vi "order-spectrum-flexlogger-test.vi"(1 "Order Settings":T2={"pulses per rev"=1, "trigger level (V)"=2.5, "max order"=64.0, "order resolution"=0.1, "window"=1, "averaging parameters"={"averaging mode"=enum."No averaging", "weighting mode"=enum."Linear", "number of averages"=1, "linear mode"=enum."One shot"}, "order ranges"=[{"start"=0.8, "stop"=1.2}, {"start"=1.8, "stop"=2.2}, {"start"=3.37, "stop"=3.77}, {"start"=3.8, "stop"=4.2}, {"start"=23.8, "stop"=24.2}]}, 4 "Noise (g rms)":dbl=0.01, 5 "Phases (deg)":dbl[](array[numeric])=[30.0, 0.0, 0.0, 0.0, 0.0], 6 "Orders":dbl[](array[numeric])=[1.0, 2.0, 3.57, 4.0, 24.0], 7 "Amplitudes (g pk)":dbl[](array[numeric])=[0.5, 0.2, 0.1, 0.05, 0.3], 8 "error in (no error)":errorcluster, 9 "Duration (s)":dbl=30.0, 10 "Ramps":T3(array[cluster]), 11 "Base RPM":dbl=3000.0) -> (0 "error out":errorcluster, 2 "True RPM":dbl[](array[numeric]), 3 "Tach RPM":dbl[](array[numeric]))   [LabVIEW 2026]
doc: "Unit-test harness for OrderSpectrumToFlexLogger.vi, fed block by block by the S&V order power spectrum chain of the NI example (Analog Tacho Process, Convert to Even Angle, Order Power Spectrum). Synthesises accel (sum of order sines, peak amplitudes, uniform noise) and a 1 ppr 0-5 V square tach (rising edge at shaft angle 0) for rpm(t) = Base RPM + sum of linear ramps, cuts it into 0.1 s blocks (5120 S @ 51.2 kS/s) and calls OrderPowerSpectrum.vi block by block like FlexLogger Process.vi does (Data In = [accel, tach], reset? TRUE on block 0). Returns NUMERIC arrays only: Values [blocks x (2 + order ranges)] = RPM, order amplitudes (g rms), Spectrum Valid, True RPM at each block centre."
uses:
  <vilib>/addons/Sound and Vibration/Order Analysis/Tach Process/OAT Analog Tacho Process (1 Tacho).vi
  <vilib>/addons/Sound and Vibration/Order Analysis/Resample Order Tracking/OAT Convert to Even Angle Signal (1 Channel).vi
  <vilib>/addons/Sound and Vibration/Order Analysis/Resample Order Tracking/OAT Order Power Spectrum (1 Channel).vi
  <vilib>/addons/Sound and Vibration/Order Analysis/Tach Process/SoundVib_TachProcess.lvlib
  <vilib>/addons/Sound and Vibration/Order Analysis/Resample Order Tracking/SoundVib_OrderTracking.lvlib
panel:
  out "Captured Raw Delta Order":dbl
  out "Captured Raw Order 0":dbl
  out "Captured Raw Magnitude":dbl[](array[numeric])
  out "Captured Plot Values":dbl[][](array[numeric])
  out "Log Values":dbl[][](array[numeric])
  in  "Capture Block":i32=100
  in  "Spectrum Display Settings":T1={"channels"=1, "plot points per block"=641, "plot in dB? (F)"=FALSE, "window ENBW (bins)"=1.5}
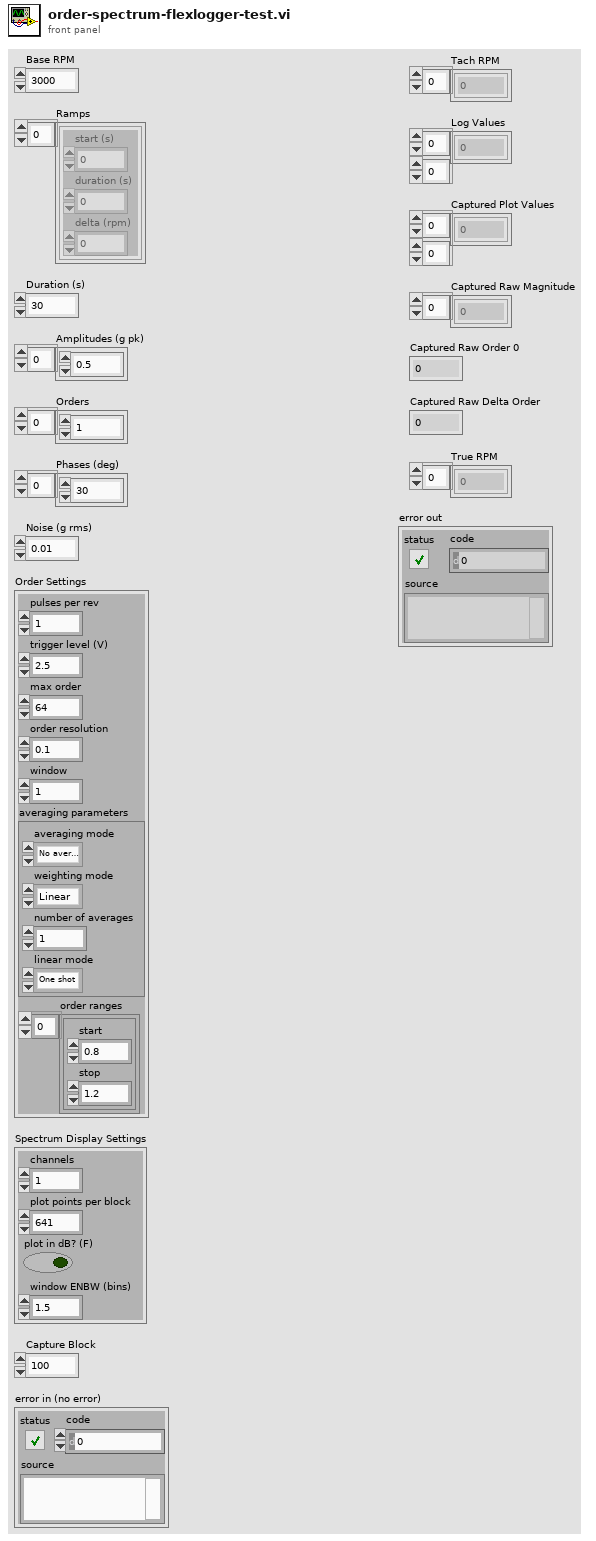
[diagram p1: front panel]
types:
  T1 = cluster{"channels":i32, "plot points per block":i32, "plot in dB? (F)":bool, "window ENBW (bins)":dbl}
  T2 = cluster{"pulses per rev":i32, "trigger level (V)":dbl, "max order":dbl, "order resolution":dbl, "window":u32, "averaging parameters":cluster{"averaging mode":enum16{"No averaging", "Vector averaging", "RMS averaging", "Peak hold"}, "weighting mode":enum16{"Linear", "Exponential"}, "number of averages":u32, "linear mode":enum16{"One shot", "Auto restart"}}, "order ranges":cluster{"start":dbl, "stop":dbl}[]}
  T3 = cluster{"start (s)":dbl, "duration (s)":dbl, "delta (rpm)":dbl}[]
  T4 = cluster{"order 0":dbl, "delta order":dbl, "magnitude":dbl[]}
  T5 = cluster{"averaging mode":enum16{"No averaging", "Vector averaging", "RMS averaging", "Peak hold"}, "weighting mode":enum16{"Linear", "Exponential"}, "number of averages":u32, "linear mode":enum16{"One shot", "Auto restart"}}
  T6 = typedef "SoundVib_TachProcess.lvlib/speed profile.ctl" = cluster{"time [s]":dbl[], "speed [RPM]":dbl[]}
  T7 = typedef "svc_Resampled Channel Info.ctl" = cluster{"channel name":string, "description":string, " channel info":T8}
  T8 = typedef "svc_Channel Info.ctl" = cluster{"sensor sensitivity":dbl, "engineering units":T9, "dB reference":dbl, "custom label":string, "weighting filter":T10, "pregain":dbl}
  T9 = typedef "svc_Engineering Units Text Ring.ctl" = u16
  T10 = typedef "svc_Weighting Filter Text Ring.ctl" = u16
  T11 = cluster{"order 0":dbl, "delta order":dbl, "magnitude":dbl[]}[]
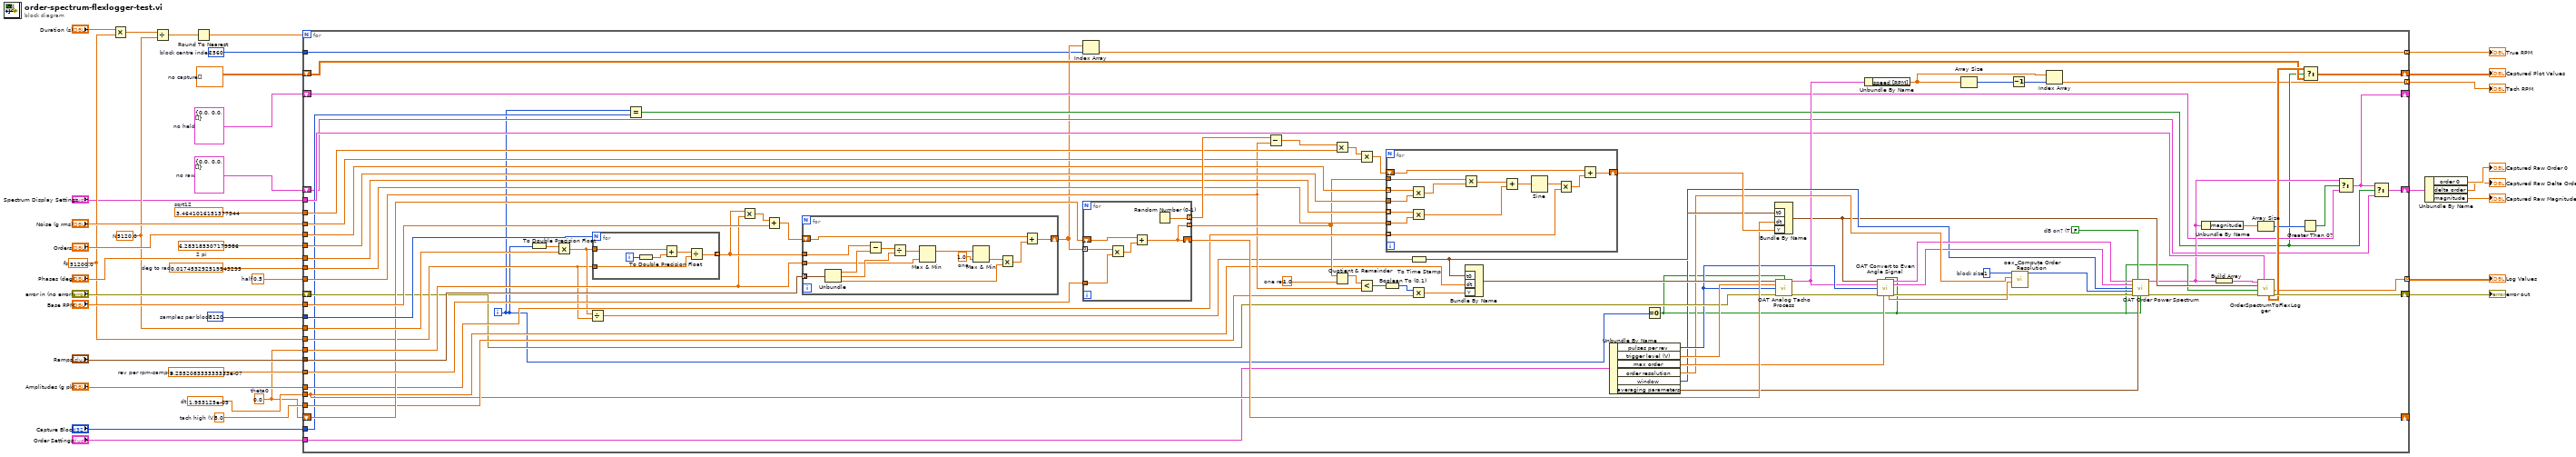
[diagram p0: block diagram]
diagram:
  w10 = T4 {"order 0"=0.0, "delta order"=0.0, "magnitude"=[]}  # no held
  w11 = T4 {"order 0"=0.0, "delta order"=0.0, "magnitude"=[]}  # no raw
  w12 = dbl[][] []  # no capture
  w17 = 2560  # block centre index
  w18 = 5.0  # tach high (V)
  w19 = 6.283185307179586  # 2 pi
  w20 = 0.017453292519943295  # deg to rad
  w21 = 0.5  # half
  w22 = 3.4641016151377544  # sqrt12
  w23 = 1.953125e-05  # dt
  w24 = 3.255208333333333e-07  # rev per rpm-sample
  w16 = 0.0  # theta0
  w25 = 5120.0  # N
  w26 = 5120  # samples per block
  w27 = 51200.0  # fs
  n1 = Multiply(x="Duration (s)", y=w27) -> (x*y=w37:dbl)
  n2 = Divide(x=w37, y=w25) -> (x/y=w36:dbl)
  n3 = Round To Nearest(number=w36) -> (nearest integer value=w13:dbl)
  n4 = for {
    N: w13 -> [_]
    shift-right: [w111] -> _
    shift-left: w16 -> [w110]
    shift-right: [w58] -> w1
    shift-left: "error in (no error)" -> [w81]
    tunnel: "Base RPM" -> [w117]
    tunnel: "Ramps" -> [w116]
    tunnel: "Amplitudes (g pk)" -> [w103]
    tunnel: "Orders" -> [w104]
    tunnel: "Phases (deg)" -> [w102]
    tunnel: "Noise (g rms)" -> [w105]
    tunnel: "Order Settings" -> [w84]
    tunnel: w27 -> [w90]
    tunnel: w26 -> [w119]
    tunnel: w25 -> [w120]
    tunnel: w24 -> [w112]
    tunnel: w23 -> [w86]
    tunnel: w22 -> [w107]
    tunnel: w21 -> [w95]
    tunnel: w20 -> [w100]
    tunnel: w19 -> [w101]
    tunnel: w18 -> [w92]
    tunnel: w17 -> [w43]
    tunnel: w16 -> [w114]
    tunnel: "Spectrum Display Settings" -> [w59]
    tunnel: "Capture Block" -> [w57]
    shift-right: [w54] -> w7
    shift-left: w12 -> [w55]
    shift-right: [w45] -> w6
    shift-left: w11 -> [w46]
    shift-right: [w48] -> _
    shift-left: w10 -> [w49]
    tunnel: [w42] -> w9 mode=indexing
    tunnel: [w41] -> w8 mode=indexing
    tunnel: [w40] -> w2 mode=indexing
    i -> [w39]
    w73 = FALSE  # dB on? (T)
    w77 = 1  # block size
    w97 = 1.0  # one rev
    n5 = To Double Precision Float(number=w39) -> (double precision float=w121:dbl)
    n6 = Multiply(x=w121, y=w120) -> (x*y=w91:dbl)
    n7 = Divide(x=w91, y=w90) -> (x/y=w89:dbl)
    n8 = for {
      N: w119 -> [_]
      tunnel: w91 -> [w161]
      tunnel: w90 -> [w158]
      tunnel: [w157] -> w115 mode=indexing
      i -> [w156]
      n9 = To Double Precision Float(number=w156) -> (double precision float=w160:dbl)
      n10 = Add(x=w161, y=w160) -> (x+y=w159:dbl)
      n11 = Divide(x=w159, y=w158) -> (x/y=w157:dbl)
    }
    n12 = Equal?(x=w39, y=w57) -> (x = y?=w47:bool)
    n13 = Multiply(x=w115, y=w114) -> (x*y=w118:dbl[])
    n14 = Add(x=w118, y=w117) -> (x+y=w113:dbl[])
    n15 = for {
      tunnel: w116 -> [w155] mode=indexing
      tunnel: w115 -> [w154]
      tunnel: w114 -> [w149]
      shift-right: [w142] -> w44
      shift-left: w113 -> [w144]
      w147 = 1.0  # one
      n16 = Unbundle(w155) -> ("start (s)"=w153:dbl, "duration (s)"=w151:dbl, "delta (rpm)"=w145:dbl)
      n17 = Subtract(x=w154, y=w153) -> (x-y=w152:dbl[])
      n18 = Divide(x=w152, y=w151) -> (x/y=w150:dbl[])
      n19 = Max & Min(x=w150, y=w149) -> (max(x,y)=w148:dbl[])  [unwired: 1 out]
      n20 = Max & Min(x=w148, y=w147) -> (min(x,y)=w146:dbl[])  [unwired: 1 out]
      n21 = Multiply(x=w146, y=w145) -> (x*y=w143:dbl[])
      n22 = Add(x=w144, y=w143) -> (x+y=w142:dbl[])
    }
    n23 = Index Array(array=w44, index=w43) -> (element=w40:dbl)
    n24 = for {
      tunnel: w44 -> [w141] mode=indexing
      tunnel: w112 -> [w140]
      shift-right: [w137] -> w111
      shift-left: w110 -> [w139]
      tunnel: [w137] -> w98 mode=indexing
      tunnel: [w136] -> w109 mode=indexing
      n25 = Multiply(x=w141, y=w140) -> (x*y=w138:dbl)
      n26 = Add(x=w139, y=w138) -> (x+y=w137:dbl)
      n27 = Random Number (0-1)() -> (number: 0 to 1=w136:dbl)
    }
    n28 = Subtract(x=w109, y=w95) -> (x-y=w108:dbl[])
    n29 = Multiply(x=w108, y=w107) -> (x*y=w106:dbl[])
    n30 = Quotient & Remainder(x=w98, y=w97) -> (x-y*floor(x/y)=w96:dbl[])  [unwired: 1 out]
    n31 = Multiply(x=w106, y=w105) -> (x*y=w99:dbl[])
    n32 = Less?(x=w96, y=w95) -> (x < y?=w94:bool[])
    n33 = Boolean To (0,1)(Boolean=w94) -> (0, 1=w93:i16[])
    n34 = for {
      tunnel: w104 -> [w135] mode=indexing
      tunnel: w103 -> [w125] mode=indexing
      tunnel: w102 -> [w131] mode=indexing
      tunnel: w98 -> [w133]
      tunnel: w101 -> [w134]
      tunnel: w100 -> [w130]
      shift-right: [w122] -> w88
      shift-left: w99 -> [w124]
      n35 = Multiply(x=w135, y=w134) -> (x*y=w132:dbl)
      n36 = Multiply(x=w131, y=w130) -> (x*y=w128:dbl)
      n37 = Multiply(x=w133, y=w132) -> (x*y=w129:dbl[])
      n38 = Add(x=w129, y=w128) -> (x+y=w127:dbl[])
      n39 = Sine(x=w127) -> (sin(x)=w126:dbl[])
      n40 = Multiply(x=w126, y=w125) -> (x*y=w123:dbl[])
      n41 = Add(x=w124, y=w123) -> (x+y=w122:dbl[])
    }
    n42 = Multiply(x=w93, y=w92) -> (x*y=w85:dbl[])
    n43 = To Time Stamp(1:w89) -> (0:w87:timestamp)
    n44 = Bundle By Name("t0"=w87, "dt"=w86, "Y"=w85) -> (w83:waveform(dbl))  [unwired: 1 in]
    n45 = Unbundle By Name(w84) -> ("pulses per rev"=w80:i32, "trigger level (V)"=w82:dbl, "max order"=w79:dbl, "order resolution"=w76:dbl, "window"=w71:u32, "averaging parameters"=w68:T5)
    n46 = Equal To 0?(x=w39) -> (x = 0?=w61:bool)
    n47 = Bundle By Name("t0"=w87, "dt"=w86, "Y"=w88) -> (w62:waveform(dbl))  [unwired: 1 in]
    n48 = call-poly <vilib>:"OAT Analog Tacho Process.vi"("analog tacho signal"=w83, "reset? (F)"=w61, "threshold (auto)"=w82, "pulse/revolution (1)"=w80, "error in (no error)"=w81) -> ("speed profile"=w67:T6, "error out"=w78:errorcluster)  [unwired: 6 in, 3 out]
    n49 = Unbundle By Name(w67) -> ("speed [RPM]"=w65:dbl[])
    n50 = call-poly <vilib>:"OAT Convert to Even Angle Signal.vi"("scaled signal [EU]"=w62, "reset? (F)"=w61, "speed profile"=w67, "pulse/revolution (1)"=w80, "error in (no error)"=w78, "max order (auto)"=w79) -> ("even-angle signal"=w74:cluster{"r0":dbl, "dr":dbl, "Y":dbl[]}, "even-angle channel info"=w72:T7, "actual max order"=w75:dbl, "error out"=w69:errorcluster)  [unwired: 5 in, 1 out]
    n51 = Array Size(array=w65) -> (size(s)=w66:i32)
    n52 = Decrement(x=w66) -> (x-1=w64:i32)
    n53 = call <vilib>:"oax_Compute Order Resolution.vi"("actual max order"=w75, "order resolution"=w76, "block size"=w77) -> ("block size out"=w70:i32)  [unwired: 7 in, 1 out]
    n54 = Index Array(array=w65, index=w64) -> (element=w42:dbl)
    n55 = call-poly <vilib>:"OAT Order Power Spectrum.vi"("even-angle signal"=w74, "dB on? (T)"=w73, "even-angle channel info"=w72, "window"=w71, "block size"=w70, "error in (no error)"=w69, "averaging parameters"=w68, "restart averaging? (F)"=w61) -> ("order power spectrum"=w51:T4, "error out"=w60:errorcluster)  [unwired: 1 in, 5 out]
    n56 = Unbundle By Name(w51) -> ("magnitude"=w53:dbl[])
    n57 = Build Array(w51) -> (w63:T11)
    n58 = Array Size(array=w53) -> (size(s)=w52:i32)
    n59 = call "OrderSpectrumToFlexLogger.vi"("Spectrum Display Settings"=w59, "error in (no error)"=w60, "reset? (F)"=w61, "Timing Reference"=w62, "order power spectra"=w63) -> ("error out"=w58:errorcluster, "Log Values"=w41:dbl[], "Plot Values"=w56:dbl[][])  [unwired: 2 in, 2 out]
    n60 = Greater Than 0?(x=w52) -> (x > 0?=w50:bool)
    n61 = Select(t=w56, s=w47, f=w55) -> (s? t:f=w54:dbl[][])
    n62 = Select(t=w51, s=w50, f=w49) -> (s? t:f=w48:T4)
    n63 = Select(t=w48, s=w47, f=w46) -> (s? t:f=w45:T4)
  }
  "Tach RPM" <- w9
  "Log Values" <- w8
  "Captured Plot Values" <- w7
  "True RPM" <- w2
  "error out" <- w1
  n64 = Unbundle By Name(w6) -> ("order 0"=→"Captured Raw Order 0":dbl, "delta order"=→"Captured Raw Delta Order":dbl, "magnitude"=→"Captured Raw Magnitude":dbl[])
